vi "FlatToRichauth_SubscribeLoginResponse.vi"(5 "OutputClusterType":T1, 11 "InputCluster":T3) -> (3 "OutputCluster":T1)   [LabVIEW 2020, in "grpc-auth_client.lvlib"]
uses:
  grpc-auth_client.lvlib
  auth_SubscribeLoginResponse_Flat.ctl
  auth_LoginStatus.ctl
  auth_SubscribeLoginResponse.ctl
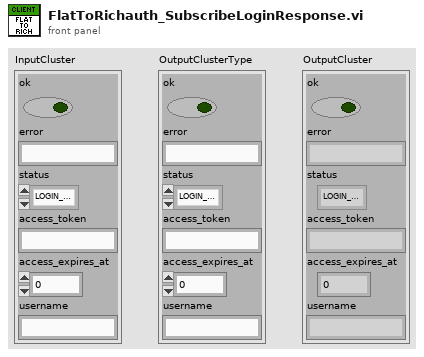
[diagram p1: front panel]
types:
  T1 = typedef "grpc-auth_client.lvlib/auth_SubscribeLoginResponse.ctl" = cluster{"ok":bool, "error":string, "status":T2, "access_token":string, "access_expires_at":i64, "username":string}
  T2 = typedef "grpc-auth_client.lvlib/auth_LoginStatus.ctl" = enum32{"LOGIN_STATUS_PENDING", "LOGIN_STATUS_READY", "LOGIN_STATUS_EXPIRED", "LOGIN_STATUS_USED", "LOGIN_STATUS_INVALID"}
  T3 = typedef "grpc-auth_client.lvlib/auth_SubscribeLoginResponse_Flat.ctl" = cluster{"ok":bool, "error":string, "status":T2, "access_token":string, "access_expires_at":i64, "username":string}
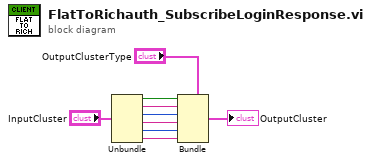
[diagram p0: block diagram]
diagram:
  n1 = Unbundle "Unbundle"("InputCluster") -> ("ok"=w6:bool, "error"=w5:string, "status"=w4:T2, "access_token"=w3:string, "access_expires_at"=w2:i64, "username"=w1:string)
  n2 = Bundle "Bundle"(cluster="OutputClusterType", "ok"=w6, "error"=w5, "status"=w4, "access_token"=w3, "access_expires_at"=w2, "username"=w1) -> (→"OutputCluster":T1)
